vi "Linear Measurement Panel Close.vi"(8 "error in (no error)":errorcluster caption="错误输入（无错误）", 10 "Linear Measurement Module ID":i32, 11 "Data Viewer 输入":refnum<class "Data Viewer.lvclass">) -> (0 "error out":errorcluster caption="错误输出", 3 "Data Viewer 输出":refnum<class "Data Viewer.lvclass">)   [LabVIEW 2020, in "Data Viewer.lvlib" / "Data Viewer.lvclass"]
uses:
  Data Viewer.lvclass
  Data Viewer.lvclass/Data Viewer.ctl
  Data Viewer.lvlib
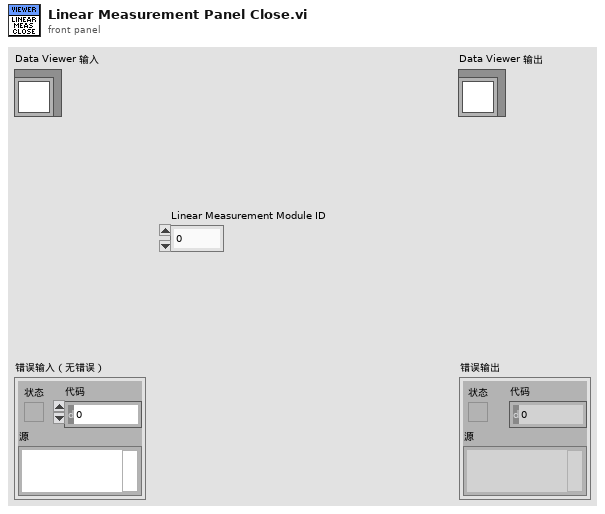
[diagram p1: front panel]
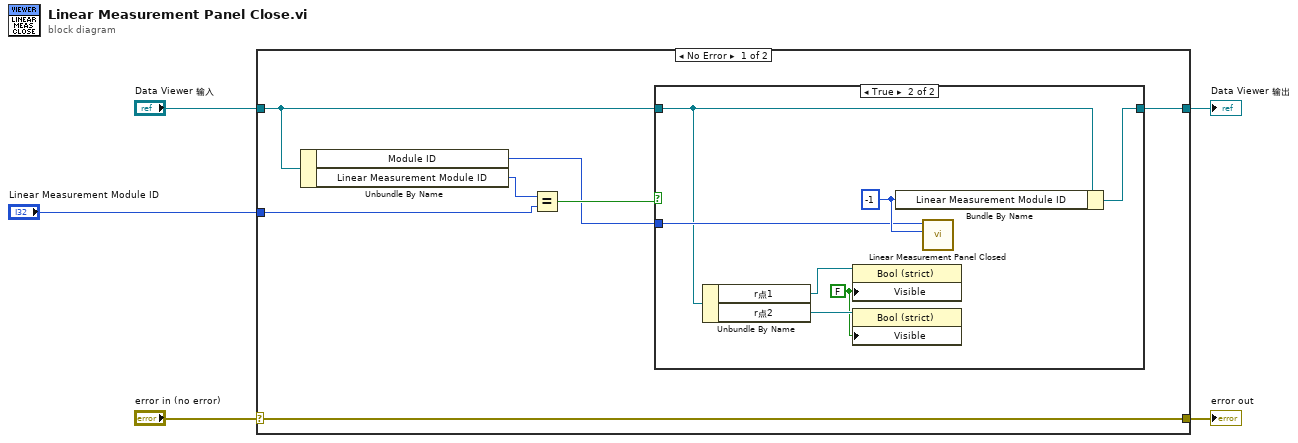
[diagram p0: block diagram]
diagram:
  n1 = case shown="No Error" "error in (no error)" {
    selector: "error in (no error)" -> [w12 w22]
    tunnel: [w12 w22] -> w4
    tunnel: [w9 w21] -> w2
    tunnel: "Data Viewer 输入" -> [w11 w21]
    tunnel: "Linear Measurement Module ID" -> [w10 _]
    frame No Error {
      n2 = Unbundle By Name(w11) -> ("Module ID"=w6:i32, "Linear Measurement Module ID"=w8:i32)
      n3 = Equal?(x=w8, y=w10) -> (x = y?=w7:bool)
      n4 = case shown="True" w7 {
        tunnel: w11 -> [w13 w17]
        tunnel: [w13 w20] -> w9
        tunnel: w6 -> [_ w18]
        frame False {
        }
        frame True {
          w14 = FALSE ("可见")
          w19 = -1 ("Linear Measurement Module ID")
          n5 = Unbundle By Name(w17) -> ("r点1"=w15:refnum<vi>, "r点2"=w16:refnum<vi>)
          n6 = property class="Bool (strict)"(reference=w15, "Visible"=w14) -> ()  [unwired: 1 in, 2 out]
          n7 = property class="Bool (strict)"(reference=w16, "Visible"=w14) -> ()  [unwired: 1 in, 2 out]
          n8 = Bundle By Name(cluster=w17, "Linear Measurement Module ID"=w19) -> (w20:refnum<class "Data Viewer.lvclass">)
          n9 = call "Linear Measurement Panel Closed.vi"("Linear Measurement Module ID"=w19, "Module ID"=w18) -> ()  [unwired: 9 in, 1 out]
        }
      }
    }
    frame Error {
    }
  }
  "error out" <- w4
  "Data Viewer 输出" <- w2
